vi "Select Bus.vi"(11 "Modes":T1) -> (0 "error out":errorcluster, 3 "Array":refnum<class "Bus_Access.lvclass">[](array[class]))   [LabVIEW 2021]
uses:
  Demo Mode.ctl
  <vilib>/TSA/Omni-Bus/Omni-Bus/Bus Access/Bus_Access.lvclass
  <vilib>/TSA/Omni-Bus/Local Bus/Local Bus.lvclass
  C:/Program Files (x86)/National Instruments/LabVIEW 2021/vi.lib/TSA/Omni-Bus/Omni-Bus/Bus Access/Bus_Access.lvclass
  <vilib>/TSA/Omni-Bus/Local Bus/Support/Tag List Type.ctl
  <vilib>/Utility/Data Type/Type Definitions/Data Type.ctl
  <vilib>/TSA/Omni-Bus/Remap Bus/Remap Bus.lvclass
  <vilib>/TSA/Omni-Bus/Remap Bus/Support/Remap Table Type.ctl
  <vilib>/TSA/Omni-Bus/Fault-Injection Bus/Fault-Injection Bus.lvclass
  <vilib>/TSA/Scale-Bus/Scale-Bus/Scale-Bus.lvclass
  <vilib>/TSA/FPGA-Bus/FPGA-Bus.lvclass
  <vilib>/TSA/Abstract Data Classes/Abs_Types/Numeric/Abs_Numeric.lvclass
  <vilib>/TSA/CTI-Bus/Children/Serial/CTI_Serial_Bus.lvclass
  <vilib>/TSA/CTI-Bus/Channels/GPIO/DigitalOut/CTI_GPIO_DigitalOut.lvclass
  C:/Program Files (x86)/National Instruments/LabVIEW 2021/vi.lib/TSA/Abstract Data Classes/Abs_Types/Value/Abs_Value.lvclass
  <vilib>/CTI/CTI Drivers/CTI/GPIO Number.ctl
  <vilib>/CTI/CTI Drivers/CTI/GPIO Pull.ctl
  <vilib>/TSA/CTI-Bus/Channels/Analog In/CTI_AnalogIn.lvclass
  <vilib>/CTI/CTI Drivers/CTI/ADC Number.ctl
  <vilib>/TSA/DAQmx-Bus/DAQmx-Bus.lvclass
  <vilib>/TSA/Scale-Bus/Scale-Value/Linear/Scale-Value Linear.lvclass
  C:/Program Files (x86)/National Instruments/LabVIEW 2021/vi.lib/TSA/Abstract Data Classes/Abs_Types/Numeric/Abs_Numeric.lvclass
  <vilib>/TSA/Scale-Bus/Scale-Value/Thermocouple/Scale-Value Thermocouple.lvclass
  <vilib>/FPGAPlugInAG/cRIO-9053/niLvFpga_Open_cRIO-9053.vi
  <vilib>/rvi/interface/common/dynamic/niFpgaDynamicAddResources.vi
  <vilib>/rvi/interface/nirviOpenFPGA/nirviOpenFPGA.xnode
  FPGA Bitfiles/presentationdemo_FPGATarget_FPGAMain_cWYV6TbVDtY.lvbitx
  <vilib>/Utility/Data Type/NI_Data Type.lvlib
  <vilib>/CTI/CTI Drivers/CTI/CTI.lvlib
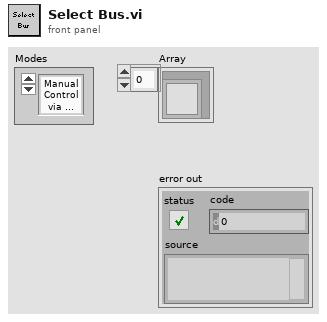
[diagram p1: front panel]
types:
  T1 = typedef "Demo Mode.ctl" = enum16{"Manual Control via Local Bus", "Software In the Loop via Local Bus", "NI USB6001 DAQ via DAQmx - Without Aliasing", "NI USB6001 DAQ via DAQmx - With Aliasing", "NI cRIO FPGA via TCP", "Community Training Initiative Raspberry Pi Pico", "NI USB6001 DAQ via DAQmx with Fault Insertion", "Mixed Devices"}
  T2 = typedef "Local Bus.lvclass/Tag List Type.ctl" = cluster{"Tag":string, "Type":T3}
  T3 = typedef "NI_Data Type.lvlib/Data Type.ctl" = enum8{"Invalid Type", "Void", "I8", "I16", "I32", "I64", "U8", "U16", "U32", "U64", "Single Float", "Double Float", "Extended Float", "Single Complex", "Double Complex", "Extended Complex", "Enum U8", "Enum U16", "Enum U32", "Enum U64", "Single Float With Unit", "Double Float With Unit", "Extended Float With Unit", "Single Complex with Unit", "Double Complex with Unit", "Extended Complex with Unit", "Boolean", "String", "Path", "Picture", "Tag", "Array", "Cluster", "Variant", "LV Variant", "Waveform", "Timestamp", "Digital Waveform", "Digital Data", "ExpressData", "Refnum", "External Data", "VI", "Poly VI", "LabVIEW Class Instance", "Fixed Point", "Set Collection", "Map Collection"}
  T4 = typedef "Remap Bus.lvclass/Remap Table Type.ctl" = cluster{"Old Tag":string, "New Tag":string}
  T5 = enum16{"Set Read Calculate Write", "Set Write Calculate Read"}
  T6 = cluster{"Tags":string[], "Scale":refnum<class "Abs_Numeric.lvclass">}
  T7 = typedef "CTI.lvlib/ADC Number.ctl" = i8
  T8 = typedef "CTI.lvlib/GPIO Pull.ctl" = enum16{"None", "Up", "Down", "Both"}
  T9 = typedef "CTI.lvlib/GPIO Number.ctl" = i8
  T10 = cluster{"Tags":string[], "Scale":refnum<class "Abs_Numeric.lvclass">}[]
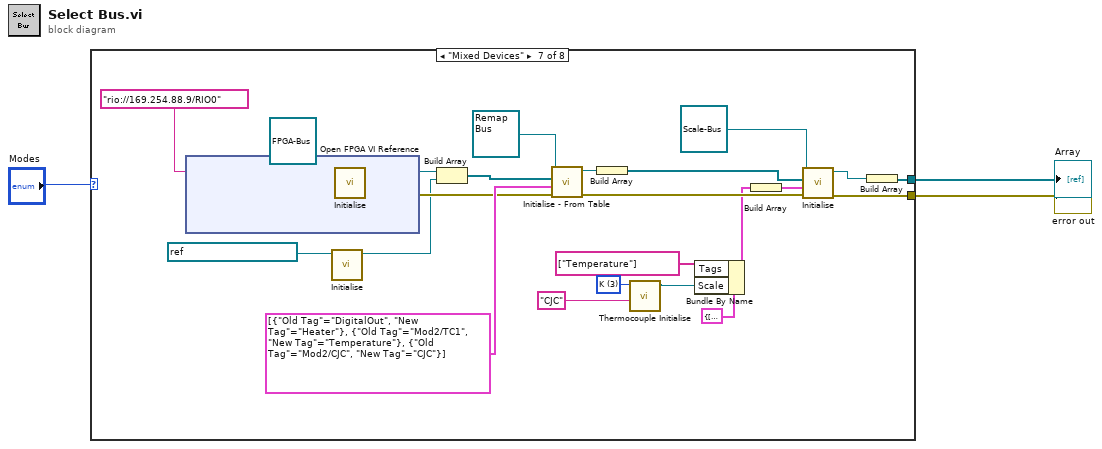
[diagram p0: block diagram]
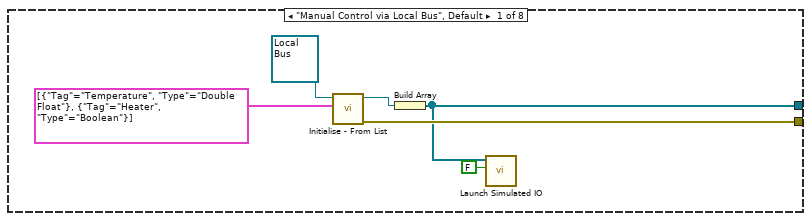
[diagram p2: hidden frame]
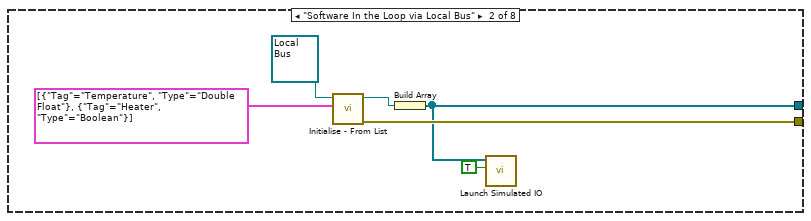
[diagram p3: hidden frame]
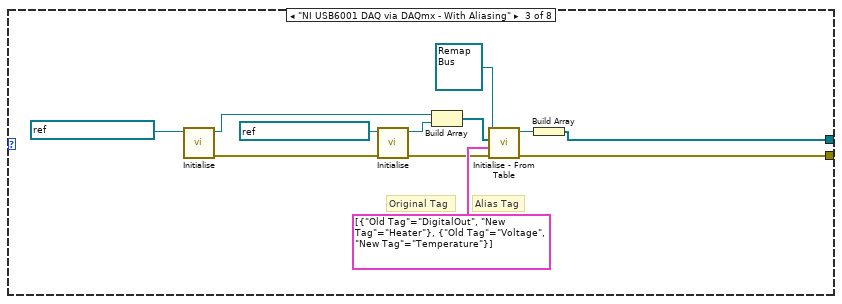
[diagram p4: hidden frame]
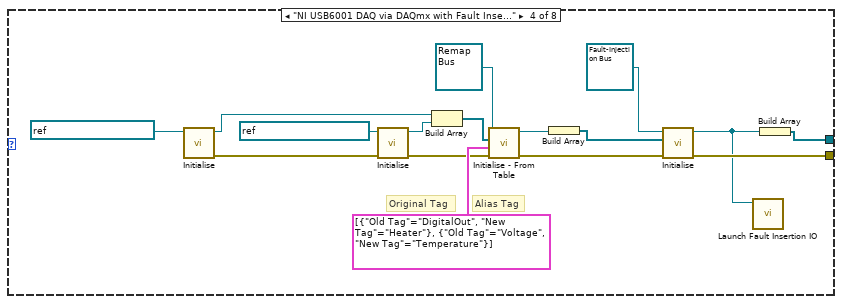
[diagram p5: hidden frame]
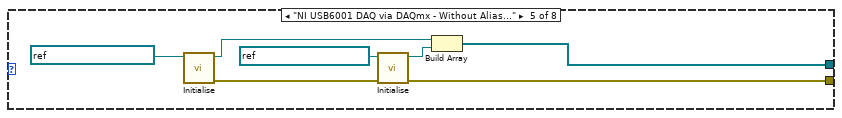
[diagram p6: hidden frame]
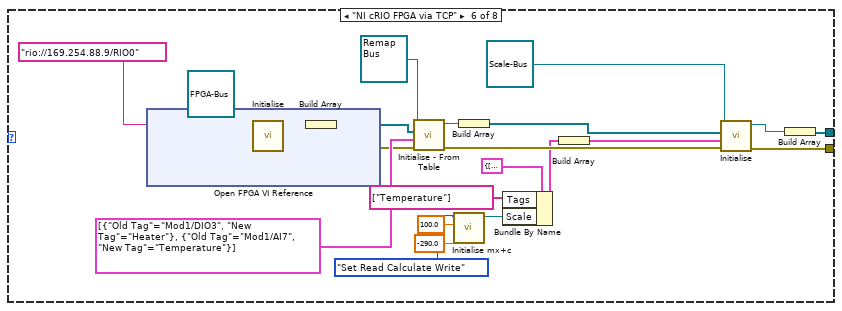
[diagram p7: hidden frame]
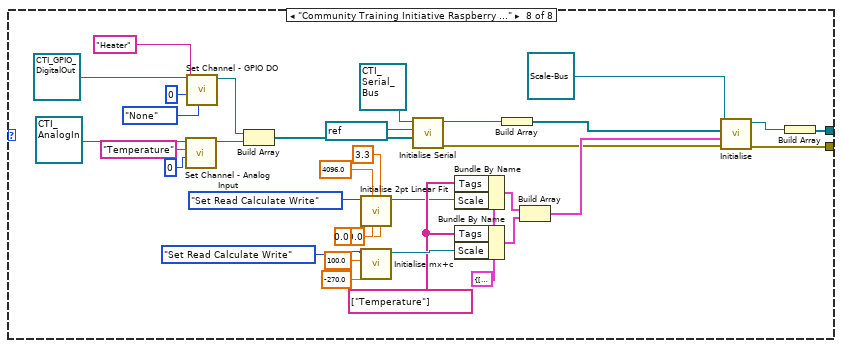
[diagram p8: hidden frame]
diagram:
  n1 = case shown="\"Mixed Devices\"" "Modes" {
    tunnel: [w9 w15 w26 w30 w45 w70 w95 w131] -> w1
    tunnel: [w8 w14 w27 w43 w44 w71 w96 w132] -> w2
    frame "Manual Control via Local Bus", Default {
      n2 = call <vilib>:"Initialise - From List.vi"("Tag List"=T2[] [{"Tag"="Temperature", "Type"=enum."Double Float"}, {"Tag"="Heater", "Type"=enum."Boolean"}], "Local Bus in"=refnum<class "Local Bus.lvclass"> refnum) -> ("error out"=w9:errorcluster, "Local Bus out"=w7:refnum<class "Local Bus.lvclass">)  [unwired: 8 in]
      n3 = Build Array(w7) -> (w8:refnum<class "Local Bus.lvclass">[])
      n4 = call "Launch Simulated IO.vi"("Sim"=FALSE, "Bus Access"=w8) -> ()  [unwired: 10 in]
    }
    frame "Software In the Loop via Local Bus" {
      n5 = call <vilib>:"Initialise - From List.vi"("Tag List"=T2[] [{"Tag"="Temperature", "Type"=enum."Double Float"}, {"Tag"="Heater", "Type"=enum."Boolean"}], "Local Bus in"=refnum<class "Local Bus.lvclass"> refnum) -> ("error out"=w15:errorcluster, "Local Bus out"=w13:refnum<class "Local Bus.lvclass">)  [unwired: 8 in]
      n6 = Build Array(w13) -> (w14:refnum<class "Local Bus.lvclass">[])
      n7 = call "Launch Simulated IO.vi"("Sim"=TRUE, "Bus Access"=w14) -> ()  [unwired: 10 in]
    }
    frame "NI USB6001 DAQ via DAQmx - With Aliasing" {
      # "Alias Tag"
      # "Original Tag"
      n8 = call <vilib>:"Initialise.vi"("DAQmx Task"=refnum<k21> "Analog Input Task") -> ("error out"=w17:errorcluster, "DAQmx-Bus out"=w18:refnum<class "DAQmx-Bus.lvclass">)  [unwired: 9 in]
      n9 = call <vilib>:"Initialise.vi"("error in (no error)"=w17, "DAQmx Task"=refnum<k21> "Digital Output Task") -> ("error out"=w16:errorcluster, "DAQmx-Bus out"=w21:refnum<class "DAQmx-Bus.lvclass">)  [unwired: 8 in]
      n10 = Build Array(w18, w21) -> (w20:refnum<class "DAQmx-Bus.lvclass">[])
      n11 = call <vilib>:"Initialise - From Table.vi"("error in (no error)"=w16, "Remapped Tags"=T4[] [{"Old Tag"="DigitalOut", "New Tag"="Heater"}, {"Old Tag"="Voltage", "New Tag"="Temperature"}], "Buses"=w20, "Remap Bus in"=refnum<class "Remap Bus.lvclass"> refnum) -> ("error out"=w26:errorcluster, "Remap Bus out"=w25:refnum<class "Remap Bus.lvclass">)  [unwired: 6 in]
      n12 = Build Array(w25) -> (w27:refnum<class "Remap Bus.lvclass">[])
    }
    frame "NI USB6001 DAQ via DAQmx with Fault Insertion" {
      # "Alias Tag"
      # "Original Tag"
      n13 = call <vilib>:"Initialise.vi"("DAQmx Task"=refnum<k21> "Analog Input Task") -> ("error out"=w35:errorcluster, "DAQmx-Bus out"=w36:refnum<class "DAQmx-Bus.lvclass">)  [unwired: 9 in]
      n14 = call <vilib>:"Initialise.vi"("error in (no error)"=w35, "DAQmx Task"=refnum<k21> "Digital Output Task") -> ("error out"=w34:errorcluster, "DAQmx-Bus out"=w39:refnum<class "DAQmx-Bus.lvclass">)  [unwired: 8 in]
      n15 = Build Array(w36, w39) -> (w38:refnum<class "DAQmx-Bus.lvclass">[])
      n16 = call <vilib>:"Initialise - From Table.vi"("error in (no error)"=w34, "Remapped Tags"=T4[] [{"Old Tag"="DigitalOut", "New Tag"="Heater"}, {"Old Tag"="Voltage", "New Tag"="Temperature"}], "Buses"=w38, "Remap Bus in"=refnum<class "Remap Bus.lvclass"> refnum) -> ("error out"=w31:errorcluster, "Remap Bus out"=w33:refnum<class "Remap Bus.lvclass">)  [unwired: 6 in]
      n17 = Build Array(w33) -> (w29:refnum<class "Remap Bus.lvclass">[])
      n18 = call <vilib>:"Initialise.vi"("error in (no error)"=w31, "Buses"=w29, "Fault-Injection Bus in"=refnum<class "Fault-Injection Bus.lvclass"> refnum) -> ("error out"=w30:errorcluster, "Fault-Injection Bus out"=w28:refnum<class "Fault-Injection Bus.lvclass">)  [unwired: 7 in]
      n19 = call "Launch Fault Insertion IO.vi"("Fault-Injection Bus"=w28) -> ()  [unwired: 11 in]
      n20 = Build Array(w28) -> (w43:refnum<class "Fault-Injection Bus.lvclass">[])
    }
    frame "NI USB6001 DAQ via DAQmx - Without Aliasing" {
      n21 = call <vilib>:"Initialise.vi"("DAQmx Task"=refnum<k21> "Analog Input Task") -> ("error out"=w46:errorcluster, "DAQmx-Bus out"=w47:refnum<class "DAQmx-Bus.lvclass">)  [unwired: 9 in]
      n22 = call <vilib>:"Initialise.vi"("error in (no error)"=w46, "DAQmx Task"=refnum<k21> "Digital Output Task") -> ("error out"=w45:errorcluster, "DAQmx-Bus out"=w49:refnum<class "DAQmx-Bus.lvclass">)  [unwired: 8 in]
      n23 = Build Array(w47, w49) -> (w44:refnum<class "DAQmx-Bus.lvclass">[])
    }
    frame "NI cRIO FPGA via TCP" {
      n24 = xnode "Open FPGA VI Reference"("resource name"=tag "rio://169.254.88.9/RIO0") -> ("FPGA VI Reference Out"=w67:refnum<k20>, "error out"=w68:errorcluster)  [unwired: 1 in]
      n25 = call <vilib>:"Initialise.vi"("error in (no error)"=w68, "FPGA Interface"=w67, "FPGA-Bus in"=refnum<class "FPGA-Bus.lvclass"> refnum) -> ("error out"=w61:errorcluster, "FPGA-Bus out"=w73:refnum<class "FPGA-Bus.lvclass">)  [unwired: 7 in]
      n26 = Build Array(w73) -> (w62:refnum<class "FPGA-Bus.lvclass">[])
      n27 = call <vilib>:"Initialise - From Table.vi"("error in (no error)"=w61, "Remapped Tags"=T4[] [{"Old Tag"="Mod1/DIO3", "New Tag"="Heater"}, {"Old Tag"="Mod1/AI7", "New Tag"="Temperature"}], "Buses"=w62, "Remap Bus in"=refnum<class "Remap Bus.lvclass"> refnum) -> ("error out"=w60:errorcluster, "Remap Bus out"=w65:refnum<class "Remap Bus.lvclass">)  [unwired: 6 in]
      n28 = call <vilib>:"Initialise mx+c.vi"("c"=-290.0, "m"=100.0, "Scaling Mode"=T5."Set Read Calculate Write") -> ("Scale-Value Linear out"=w53:refnum<class "Scale-Value Linear.lvclass">)  [unwired: 7 in, 1 out]
      n29 = Build Array(w65) -> (w59:refnum<class "Remap Bus.lvclass">[])
      n30 = Bundle By Name(cluster=T6 {"Tags"=[], "Scale"=refnum} ("Cluster"), "Tags"=string[] ["Temperature"], "Scale"=w53) -> (w58:T6)
      n31 = Build Array(w58) -> (w57:T10)
      n32 = call <vilib>:"Initialise.vi"("error in (no error)"=w60, "Tag to Scale"=w57, "Buses"=w59, "Scale-Bus in"=refnum<class "Scale-Bus.lvclass"> refnum) -> ("error out"=w70:errorcluster, "Scale-Bus out"=w72:refnum<class "Scale-Bus.lvclass">)  [unwired: 6 in]
      n33 = Build Array(w72) -> (w71:refnum<class "Scale-Bus.lvclass">[])
    }
    frame "Mixed Devices" {
      w76 = u16 3 items=["B", "E", "J", "K", "R", "S", "T", "N"] ("ThermocoupleType")
      n34 = xnode "Open FPGA VI Reference"("resource name"=tag "rio://169.254.88.9/RIO0") -> ("FPGA VI Reference Out"=w92:refnum<k20>, "error out"=w93:errorcluster)  [unwired: 1 in]
      n35 = call <vilib>:"Initialise.vi"("DAQmx Task"=refnum<k21> "Digital Output Task") -> ("DAQmx-Bus out"=w79:refnum<class "DAQmx-Bus.lvclass">)  [unwired: 9 in, 1 out]
      n36 = call <vilib>:"Initialise.vi"("error in (no error)"=w93, "FPGA Interface"=w92, "FPGA-Bus in"=refnum<class "FPGA-Bus.lvclass"> refnum) -> ("error out"=w86:errorcluster, "FPGA-Bus out"=w98:refnum<class "FPGA-Bus.lvclass">)  [unwired: 7 in]
      n37 = Build Array(w98, w79) -> (w87:refnum<class "Bus_Access.lvclass">[])
      n38 = call <vilib>:"Initialise - From Table.vi"("error in (no error)"=w86, "Remapped Tags"=T4[] [{"Old Tag"="DigitalOut", "New Tag"="Heater"}, {"Old Tag"="Mod2/TC1", "New Tag"="Temperature"}, {"Old Tag"="Mod2/CJC", "New Tag"="CJC"}], "Buses"=w87, "Remap Bus in"=refnum<class "Remap Bus.lvclass"> refnum) -> ("error out"=w85:errorcluster, "Remap Bus out"=w90:refnum<class "Remap Bus.lvclass">)  [unwired: 6 in]
      n39 = Build Array(w90) -> (w84:refnum<class "Remap Bus.lvclass">[])
      n40 = call <vilib>:"Thermocouple Initialise.vi"("CJC degC Temp Tag"="CJC", "ThermocoupleType"=w76) -> ("Scale-Value Thermocouple out"=w77:refnum<class "Scale-Value Thermocouple.lvclass">)  [unwired: 8 in, 1 out]
      n41 = Bundle By Name(cluster=T6 {"Tags"=[], "Scale"=refnum} ("Cluster"), "Tags"=string[] ["Temperature"], "Scale"=w77) -> (w83:T6)
      n42 = Build Array(w83) -> (w82:T10)
      n43 = call <vilib>:"Initialise.vi"("error in (no error)"=w85, "Tag to Scale"=w82, "Buses"=w84, "Scale-Bus in"=refnum<class "Scale-Bus.lvclass"> refnum) -> ("error out"=w95:errorcluster, "Scale-Bus out"=w97:refnum<class "Scale-Bus.lvclass">)  [unwired: 6 in]
      n44 = Build Array(w97) -> (w96:refnum<class "Scale-Bus.lvclass">[])
    }
    frame "Community Training Initiative Raspberry Pi Pico" {
      w123 = string[] ["Temperature"] ("Tags")
      w125 = T6 {"Tags"=[], "Scale"=refnum} ("Cluster")
      n45 = call <vilib>:"Set Channel - Analog Input.vi"("ADC Number"=T7 0, "Tag"="Temperature", "CTI_GPIO_DigitalOut in"=refnum<class "CTI_AnalogIn.lvclass"> refnum) -> ("CTI_GPIO_DigitalOut out"=w117:refnum<class "CTI_AnalogIn.lvclass">)  [unwired: 7 in, 1 out]
      n46 = call <vilib>:"Set Channel - GPIO DO.vi"("GPIO Pull"=GPIO_Pull."None", "GPIO Number"=T9 0, "Tag"="Heater", "CTI_GPIO_DigitalOut in"=refnum<class "CTI_GPIO_DigitalOut.lvclass"> refnum ("CTI_GPIO_DigitalOut.lvclass")) -> ("CTI_GPIO_DigitalOut out"=w118:refnum<class "CTI_GPIO_DigitalOut.lvclass">)  [unwired: 6 in, 1 out]
      n47 = Build Array(w118, w117) -> (w109:refnum<class "Abs_Value.lvclass">[])
      n48 = call <vilib>:"Initialise 2pt Linear Fit.vi"("y2"=0.0, "y1"=3.3, "x2"=0.0, "x1"=4096.0, "Scaling Mode"=T5."Set Read Calculate Write") -> ("Scale-Value Linear out"=w107:refnum<class "Scale-Value Linear.lvclass">)  [unwired: 5 in, 1 out]
      n49 = call <vilib>:"Initialise mx+c.vi"("c"=-270.0, "m"=100.0, "Scaling Mode"=T5."Set Read Calculate Write") -> ("Scale-Value Linear out"=w128:refnum<class "Scale-Value Linear.lvclass">)  [unwired: 7 in, 1 out]
      n50 = call <vilib>:"Initialise Serial.vi"("Channels"=w109, "VISA resource name"=refnum<visa-resource-name> "COM3", "CTI_Serial_Bus in"=refnum<class "CTI_Serial_Bus.lvclass"> refnum) -> ("error out"=w119:errorcluster, "CTI_Serial_Bus out"=w122:refnum<class "CTI_Serial_Bus.lvclass">)  [unwired: 7 in]
      n51 = Bundle By Name(cluster=w125, "Tags"=w123, "Scale"=w107) -> (w124:T6)
      n52 = Bundle By Name(cluster=w125, "Tags"=w123, "Scale"=w128) -> (w100:T6)
      n53 = Build Array(w122) -> (w101:refnum<class "CTI_Serial_Bus.lvclass">[])
      n54 = Build Array(w124, w100) -> (w130:T10)
      n55 = call <vilib>:"Initialise.vi"("error in (no error)"=w119, "Tag to Scale"=w130, "Buses"=w101, "Scale-Bus in"=refnum<class "Scale-Bus.lvclass"> refnum) -> ("error out"=w131:errorcluster, "Scale-Bus out"=w133:refnum<class "Scale-Bus.lvclass">)  [unwired: 6 in]
      n56 = Build Array(w133) -> (w132:refnum<class "Scale-Bus.lvclass">[])
    }
  }
  "Array" <- w2
  "error out" <- w1
